vi "UI_Draw_Tile.vi"(0 "Picture":picture, 1 "Phase":bool, 5 "Rect":T2={"left"=0, "top"=0, "right"=91, "bottom"=54}, 7 "Channel":T1={"Name"="CH000", "Value"=0.0, "High Limit"=100.0, "Low Limit"=0.0, "Save"=TRUE, "Graph"=FALSE, "Scale Min"=0.0, "Scale Max"=100.0, "Unit"="%"}, 9 "Running":bool, 11 "error in":errorcluster) -> (4 "New Picture":picture, 15 "error out":errorcluster)   [LabVIEW 2026]
doc: "채널 타일 1개(디지털 인디케이터): 이름, G(그래프)/S(저장) 표시, 값+단위.\n측정 중 값 > High Limit 이면 빨강, < Low Limit 이면 파랑으로 Phase에 맞춰 점멸."
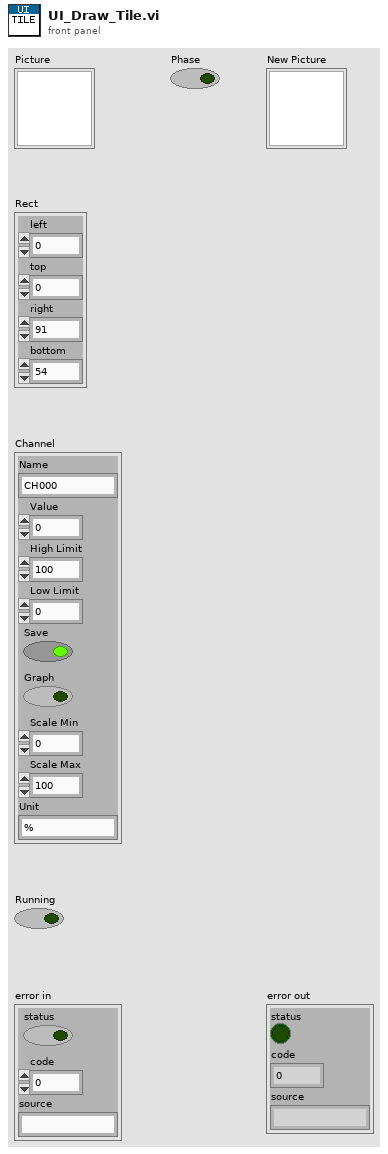
[diagram p1: front panel]
types:
  T1 = cluster{"Name":string, "Value":dbl, "High Limit":dbl, "Low Limit":dbl, "Save":bool, "Graph":bool, "Scale Min":dbl, "Scale Max":dbl, "Unit":string}
  T2 = cluster{"left":i16, "top":i16, "right":i16, "bottom":i16}
  T3 = cluster{"Font Name:":string, "Size":i16, "Strikeout?":bool, "Italic?":bool, "Underline?":bool, "Outline?":bool, "Shadow?":bool, "Bold?":bool}
  T4 = enum16{"User-specified Font", "Application Font", "System Font", "Dialog Font"}
  T5 = cluster{"horizontal":enum16{"left", "center", "right"}, "vertical":enum16{"top", "center", "bottom"}}
  T6 = cluster{"Width":u16, "Style":enum32{"Solid", "Dash", "Dot", "DashDot", "DashDotDot"}}
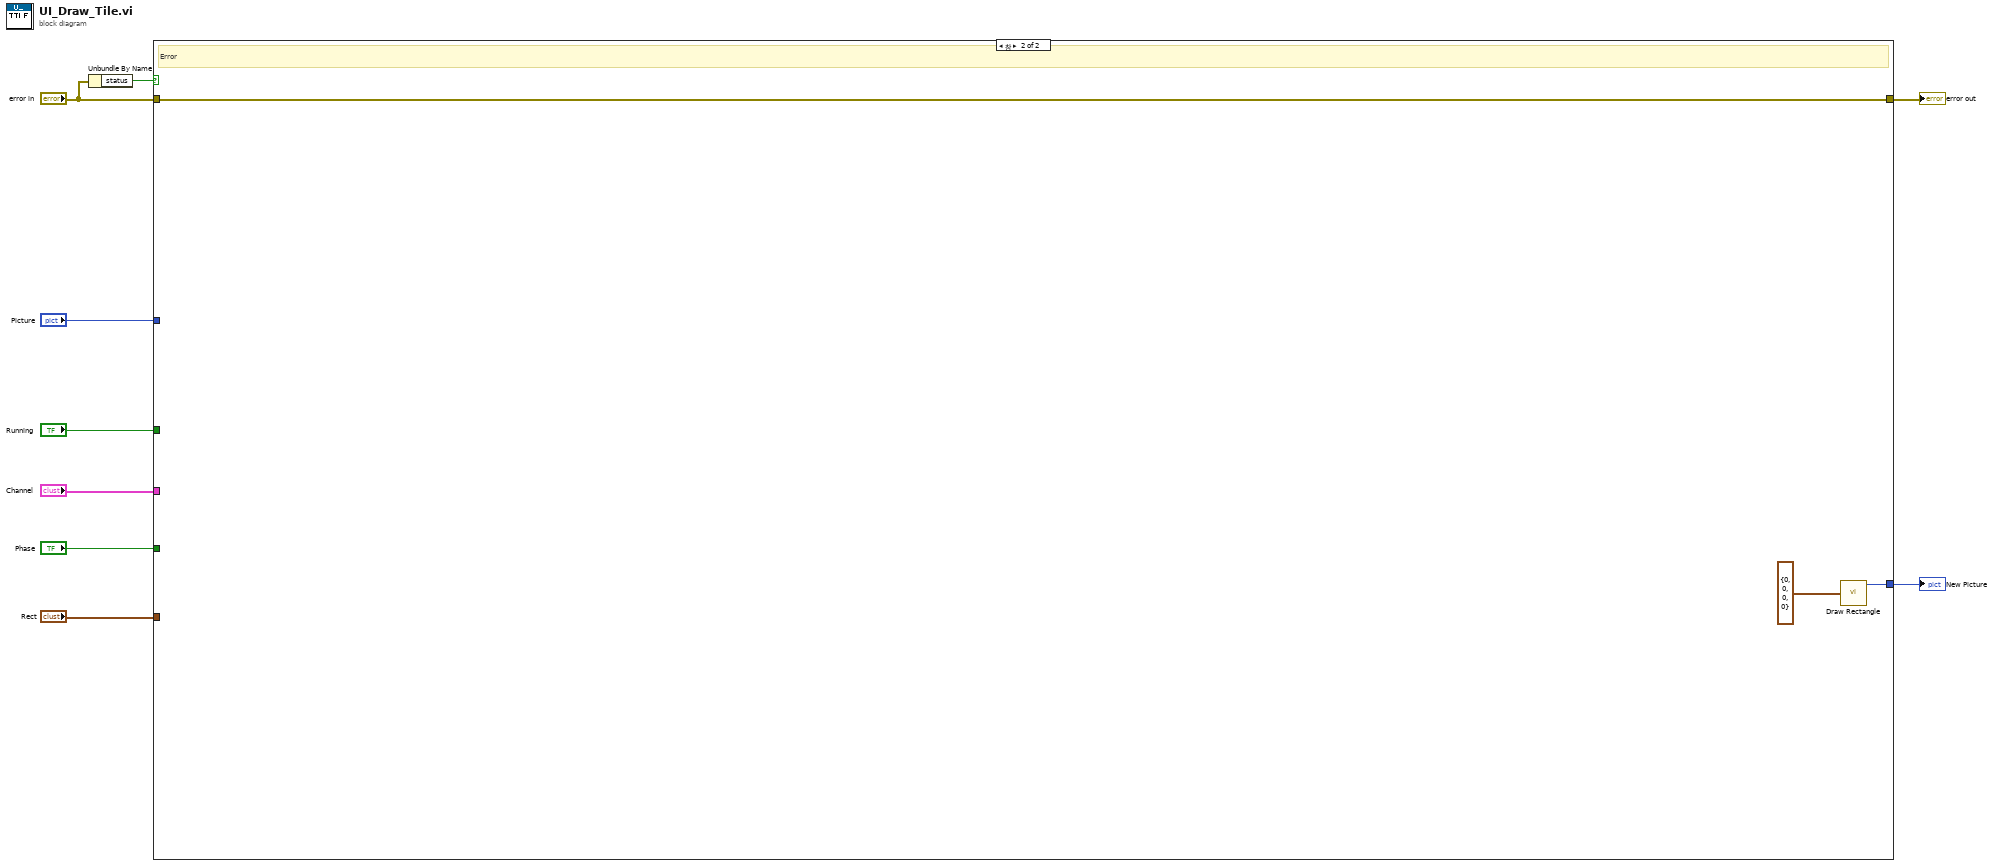
[diagram p0: block diagram]
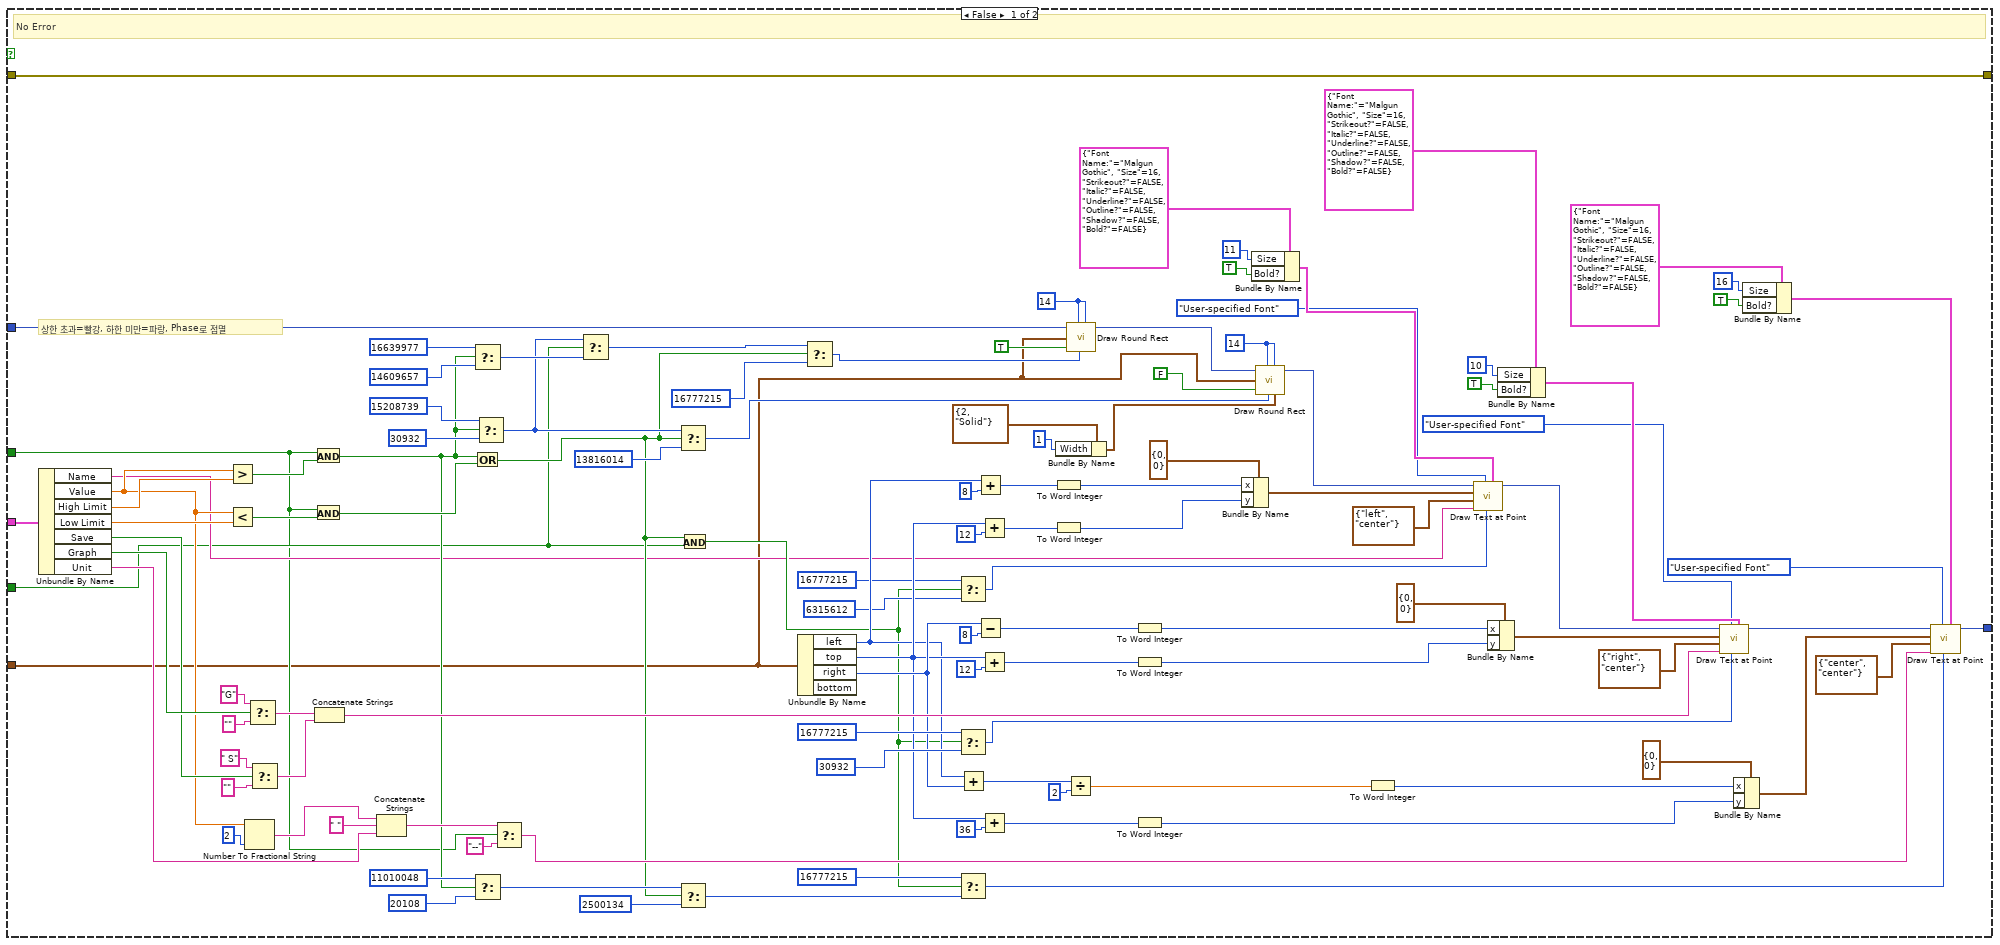
[diagram p2: hidden frame]
diagram:
  n1 = Unbundle By Name("error in") -> ("status"=w7:bool)
  n2 = case shown="참" w7 {
    tunnel: "Picture" -> [w10 _]
    tunnel: "Rect" -> [w11 _]
    tunnel: "Channel" -> [w12 _]
    tunnel: "Running" -> [w13 _]
    tunnel: "Phase" -> [w14 _]
    tunnel: "error in" -> [w15 w124]
    tunnel: [w15 w124] -> w9
    tunnel: [w123 w126] -> w8
    frame False {
      w53 = i16 14
      w50 = i16 14
      # "상한 초과=빨강, 하한 미만=파랑, Phase로 점멸"
      # "No Error"
      n3 = Unbundle By Name(w12) -> ("Name"=w16:string, "Value"=w17:dbl, "High Limit"=w18:dbl, "Low Limit"=w19:dbl, "Save"=w20:bool, "Graph"=w21:bool, "Unit"=w22:string)
      n4 = Greater?(x=w17, y=w18) -> (0:w23:bool)
      n5 = Less?(x=w17, y=w19) -> (x < y?=w25:bool)
      n6 = Number To Fractional String(number=w17, precision (6)=2) -> (F-format string=w103:string)  [unwired: 2 out]
      n7 = Select(t="G", s=w21, f="") -> (s? t:f=w79:string)
      n8 = Select(t=" S", s=w20, f="") -> (s? t:f=w82:string)
      n9 = And(x=w13, y=w23) -> (x .and. y?=w24:bool)
      n10 = And(x=w13, y=w25) -> (x .and. y?=w26:bool)
      n11 = Concatenate Strings(w79, w82) -> (w83:string)
      n12 = Concatenate Strings(w103, " ", w22) -> (w105:string)
      n13 = Select(t=u32 16639977, s=w24, f=u32 14609657) -> (s? t:f=w34:u32)
      n14 = Or(x=w24, y=w26) -> (x .or. y?=w27:bool)
      n15 = Select(t=u32 11010048, s=w24, f=u32 20108) -> (s? t:f=w43:u32)
      n16 = Select(t=u32 15208739, s=w24, f=u32 30932) -> (s? t:f=w31:u32)
      n17 = Select(t=w105, s=w13, f="--") -> (s? t:f=w107:string)
      n18 = Select(t=w31, s=w14, f=w34) -> (s? t:f=w35:u32)
      n19 = Select(t=w31, s=w27, f=u32 13816014) -> (s? t:f=w39:u32)
      n20 = Select(t=w43, s=w27, f=u32 2500134) -> (s? t:f=w45:u32)
      n21 = And(x=w27, y=w14) -> (x .and. y?=w28:bool)
      n22 = Unbundle By Name(w11) -> ("left"=w59:i16, "top"=w60:i16, "right"=w61:i16)  [unwired: 1 out]
      n23 = Select(t=w35, s=w27, f=u32 16777215) -> (s? t:f=w37:u32)
      n24 = Select(t=u32 16777215, s=w28, f=u32 6315612) -> (s? t:f=w49:u32)
      n25 = Select(t=u32 16777215, s=w28, f=u32 30932) -> (s? t:f=w94:u32)
      n26 = Select(t=u32 16777215, s=w28, f=w45) -> (s? t:f=w46:u32)
      n27 = Add(x=w59, y=w61) -> (x+y=w108:i16)
      n28 = Add(x=w59, y=i16 8) -> (x+y=w63:i16)
      n29 = Subtract(x=w61, y=i16 8) -> (x-y=w85:i16)
      n30 = Add(x=w60, y=i16 12) -> (x+y=w66:i16)
      n31 = Add(x=w60, y=i16 12) -> (x+y=w88:i16)
      n32 = Add(x=w60, y=i16 36) -> (x+y=w113:i16)
      n33 = To Word Integer(number=w63) -> (16bit integer=w64:i16)
      n34 = To Word Integer(number=w66) -> (16bit integer=w67:i16)
      n35 = Bundle By Name(cluster=T6 {"Width"=2, "Style"=enum."Solid"}, "Width"=u16 1) -> (w57:T6)
      n36 = Divide(x=w108, y=i16 2) -> (x/y=w110:dbl)
      n37 = call <vilib>:"Draw Round Rect.vi"("picture"=w10, "oval width"=w50, "rect"=w11, "fill?(F)"=TRUE, "color(black)"=w37, "oval height"=w50) -> ("new picture"=w52:picture)  [unwired: 3 in]
      n38 = To Word Integer(number=w85) -> (16bit integer=w86:i16)
      n39 = To Word Integer(number=w88) -> (16bit integer=w89:i16)
      n40 = To Word Integer(number=w113) -> (16bit integer=w114:i16)
      n41 = Bundle By Name(cluster=cluster{"x":i16, "y":i16} {"x"=0, "y"=0}, "x"=w64, "y"=w67) -> (w71:cluster{"x":i16, "y":i16})
      n42 = Bundle By Name(cluster=T3 {"Font Name:"="Malgun Gothic", "Size"=16, "Strikeout?"=FALSE, "Italic?"=FALSE, "Underline?"=FALSE, "Outline?"=FALSE, "Shadow?"=FALSE, "Bold?"=FALSE}, "Size"=i16 11, "Bold?"=TRUE) -> (w75:T3)
      n43 = call <vilib>:"Draw Round Rect.vi"("picture"=w52, "oval width"=w53, "rect"=w11, "fill?(F)"=FALSE, "color(black)"=w39, "oval height"=w53, "pen"=w57) -> ("new picture"=w58:picture)  [unwired: 2 in]
      n44 = To Word Integer(number=w110) -> (16bit integer=w111:i16)
      n45 = call <vilib>:"Draw Text at Point.vi"("[user-specified font]"=w75, "text color(black)"=w49, "desired font(Application)"=T4."User-specified Font", "text"=w16, "alignment(left, top)"=T5 {"horizontal"=enum."left", "vertical"=enum."center"}, "origin"=w71, "picture"=w58) -> ("new picture"=w76:picture)  [unwired: 3 in, 1 out]
      n46 = Bundle By Name(cluster=cluster{"x":i16, "y":i16} {"x"=0, "y"=0}, "x"=w86, "y"=w89) -> (w96:cluster{"x":i16, "y":i16})
      n47 = Bundle By Name(cluster=T3 {"Font Name:"="Malgun Gothic", "Size"=16, "Strikeout?"=FALSE, "Italic?"=FALSE, "Underline?"=FALSE, "Outline?"=FALSE, "Shadow?"=FALSE, "Bold?"=FALSE}, "Size"=i16 10, "Bold?"=TRUE) -> (w100:T3)
      n48 = call <vilib>:"Draw Text at Point.vi"("[user-specified font]"=w100, "text color(black)"=w94, "desired font(Application)"=T4."User-specified Font", "text"=w83, "alignment(left, top)"=T5 {"horizontal"=enum."right", "vertical"=enum."center"}, "origin"=w96, "picture"=w76) -> ("new picture"=w101:picture)  [unwired: 3 in, 1 out]
      n49 = Bundle By Name(cluster=cluster{"x":i16, "y":i16} {"x"=0, "y"=0}, "x"=w111, "y"=w114) -> (w118:cluster{"x":i16, "y":i16})
      n50 = Bundle By Name(cluster=T3 {"Font Name:"="Malgun Gothic", "Size"=16, "Strikeout?"=FALSE, "Italic?"=FALSE, "Underline?"=FALSE, "Outline?"=FALSE, "Shadow?"=FALSE, "Bold?"=FALSE}, "Size"=i16 16, "Bold?"=TRUE) -> (w122:T3)
      n51 = call <vilib>:"Draw Text at Point.vi"("[user-specified font]"=w122, "text color(black)"=w46, "desired font(Application)"=T4."User-specified Font", "text"=w107, "alignment(left, top)"=T5 {"horizontal"=enum."center", "vertical"=enum."center"}, "origin"=w118, "picture"=w101) -> ("new picture"=w123:picture)  [unwired: 3 in, 1 out]
    }
    frame True {
      # "Error"
      n52 = call <vilib>:"Draw Rectangle.vi"("rect"=T2 {"left"=0, "top"=0, "right"=0, "bottom"=0}) -> ("new picture"=w126:picture)  [unwired: 8 in]
    }
  }
  "New Picture" <- w8
  "error out" <- w9
